vi "CalcExpress Help.vi"   [LabVIEW 2021]
doc: "::: CalcExpress Toolkit :::\nCopyright (c) 2000-2026 Konstantin Shifershteyn. All rights reserved."
uses:
  vi.lib/addons/CalcExpress/cemisc.llb/[ce] CE component paths - Kind of Path Enum.ctl
panel:
  # "CalcExpress Toolkit\n[Help]"
types:
  T1 = enum32{"Invalid", "Standard", "Closed", "Hidden", "Minimized", "Maximized"}
  T2 = typedef "[ce] CE component paths - Kind of Path Enum.ctl" = enum16{"VIs", "FuncVIs", "Help", "Examples", "Project", "Templates"}
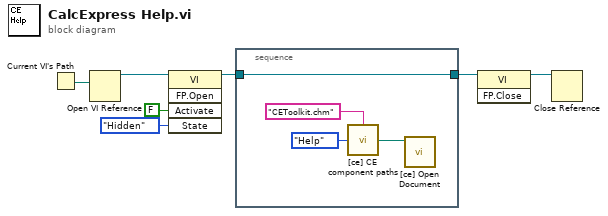
[diagram p0: block diagram]
diagram:
  n1 = Current VI's Path() -> (path=w7:path)
  n2 = Open VI Reference(vi path=w7) -> (vi reference=w4:refnum<vi>)  [unwired: 5 in, 1 out]
  n3 = invoke class="VI" method="FP.Open"(reference=w4, "Activate"=FALSE ("Activate?"), "State"=T1."Hidden") -> (reference out=w3:refnum<vi>)  [unwired: 2 in, 4 out]
  n4 = stacked-sequence {
    tunnel: w3 -> [w11]
    tunnel: [w11] -> w2
    frame #0 {
      n5 = call "[ce] CE component paths.vi"("kind of path"=[ce]_CE_component_paths_-_Kind_of_Path_Enum."Help", "append path"="CEToolkit.chm") -> ("path out"=w9:path)
      n6 = call "[ce] Open Document.vi"("file path"=w9) -> ()  [unwired: 10 in, 1 out]
    }
  }
  n7 = invoke class="VI" method="FP.Close"(reference=w2) -> (reference out=w1:refnum<vi>)  [unwired: 2 in, 2 out]
  n8 = Close Reference(reference=w1) -> ()  [unwired: 1 in, 1 out]
